vi "set VISA Timeout.vi"(8 "error in (no error)":errorcluster caption="에러 입력(에러 없음)", 10 "Timeout Value":u32, 11 "Anritsu Call Box_Implement 입력":refnum<class "Anritsu Call Box_Implement.lvclass">) -> (0 "error out":errorcluster caption="에러 출력", 3 "Anritsu Call Box_Implement 출력":refnum<class "Anritsu Call Box_Implement.lvclass">)   [LabVIEW 2023, in "ANRITSU Call Box.lvlib" / "Anritsu Call Box_Implement.lvclass"]
uses:
  Anritsu Call Box_Implement.lvclass
  Anritsu Call Box_Implement.lvclass/Anritsu Call Box_Implement.ctl
  NR/NR.lvclass
  LTE/LTE.lvclass
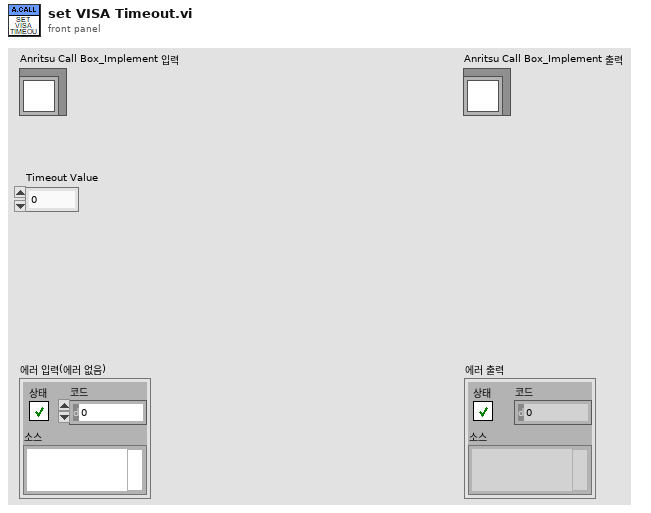
[diagram p1: front panel]
types:
  T1 = cluster{"LTE":refnum<class "LTE.lvclass">, "NR":refnum<class "NR.lvclass">}
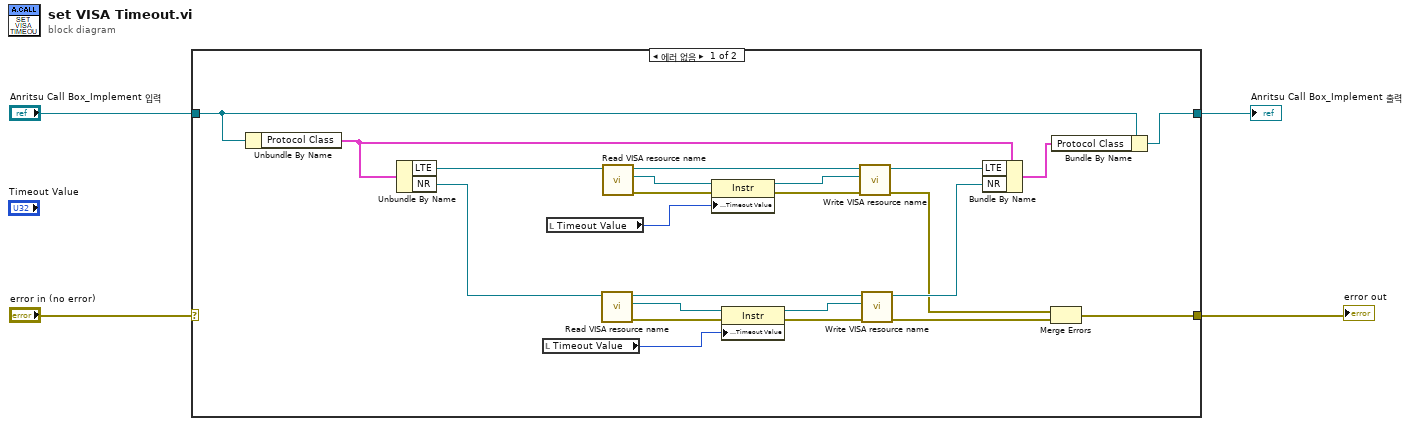
[diagram p0: block diagram]
diagram:
  n1 = case shown="에러 없음" "error in (no error)" {
    selector: "error in (no error)" -> [_ w29]
    tunnel: "Anritsu Call Box_Implement 입력" -> [w17 w28]
    tunnel: [w12 w28] -> w3
    tunnel: [w5 w29] -> w1
    frame No Error {
      n2 = Unbundle By Name(w17) -> ("Protocol Class"=w16:T1)
      n3 = Unbundle By Name(w16) -> ("LTE"=w22:refnum<class "LTE.lvclass">, "NR"=w27:refnum<class "NR.lvclass">)
      n4 = local read "Timeout Value"() -> (w23:u32)
      n5 = local read "Timeout Value"() -> (w20:u32)
      n6 = call "Read VISA resource name.vi"("NR in"=w27) -> ("error out"=w11:errorcluster, "VISA resource name"=w26:refnum<visa-resource-name>, "NR out"=w24:refnum<class "NR.lvclass">)  [unwired: 8 in]
      n7 = call "Read VISA resource name.vi"("LTE in"=w22) -> ("error out"=w9:errorcluster, "VISA resource name"=w21:refnum<visa-resource-name>, "LTE out"=w18:refnum<class "LTE.lvclass">)  [unwired: 8 in]
      n8 = property class="Instr"(reference=w21, error in=w9, "General Settings:Timeout Value"=w20) -> (reference out=w19:refnum<visa-resource-name>, error out=w8:errorcluster)
      n9 = property class="Instr"(reference=w26, error in=w11, "General Settings:Timeout Value"=w23) -> (reference out=w25:refnum<visa-resource-name>, error out=w10:errorcluster)
      n10 = call "Write VISA resource name.vi"("error in (no error)"=w8, "VISA resource name"=w19, "LTE in"=w18) -> ("error out"=w7:errorcluster, "LTE out"=w14:refnum<class "LTE.lvclass">)  [unwired: 7 in]
      n11 = call "Write VISA resource name.vi"("error in (no error)"=w10, "VISA resource name"=w25, "NR in"=w24) -> ("error out"=w6:errorcluster, "NR out"=w13:refnum<class "NR.lvclass">)  [unwired: 7 in]
      n12 = Bundle By Name(cluster=w16, "LTE"=w14, "NR"=w13) -> (w15:T1)
      n13 = Merge Errors(w7, w6) -> (w5:errorcluster)
      n14 = Bundle By Name(cluster=w17, "Protocol Class"=w15) -> (w12:refnum<class "Anritsu Call Box_Implement.lvclass">)
    }
    frame Error {
    }
  }
  "error out" <- w1
  "Anritsu Call Box_Implement 출력" <- w3
